vi "Launch Event Reporter.vi"(8 "error in (no error)":errorcluster, 11 "Volatus Core in":refnum<class "Volatus Core.lvclass">) -> (0 "error out":errorcluster, 3 "Volatus Core out":refnum<class "Volatus Core.lvclass">)   [LabVIEW 2020, in "Volatus.lvlib" / "Volatus Core.lvclass"]
uses:
  Volatus Core.lvclass
  C:/dev/lv20CE/relink/lv-volatus/Volatus/Module/Module.lvclass
  VolatusConfig/VolatusConfigElement/VolatusConfigElement.lvclass
  Module/Module.lvclass/Module.ctl
  VolatusConfig/VolatusConfigElement/VolatusConfigElement.lvclass/VolatusConfigElement.ctl
  VolatusAPI/VolatusAPI.lvclass/VolatusAPI.ctl
  Volatus Core.lvclass/Volatus Core.ctl
  VolatusConfig/VolatusConfigElement/Element.vi
  MessageQ/MessageQ.lvclass
  Module/Module.lvclass
  VolatusAPI/VolatusAPI.lvclass
  VectoEventBridge/VectoEventBridge.lvclass
  Event Reporter Module/Event Reporter Module.lvclass
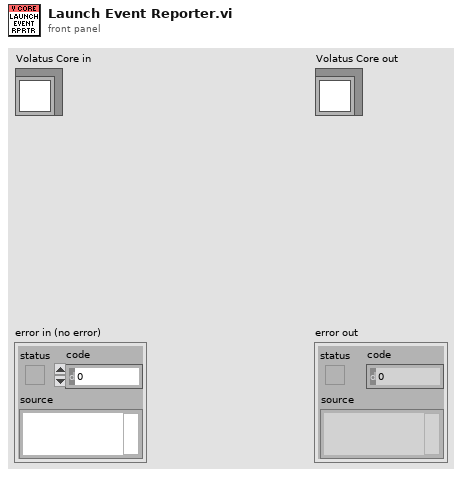
[diagram p1: front panel]
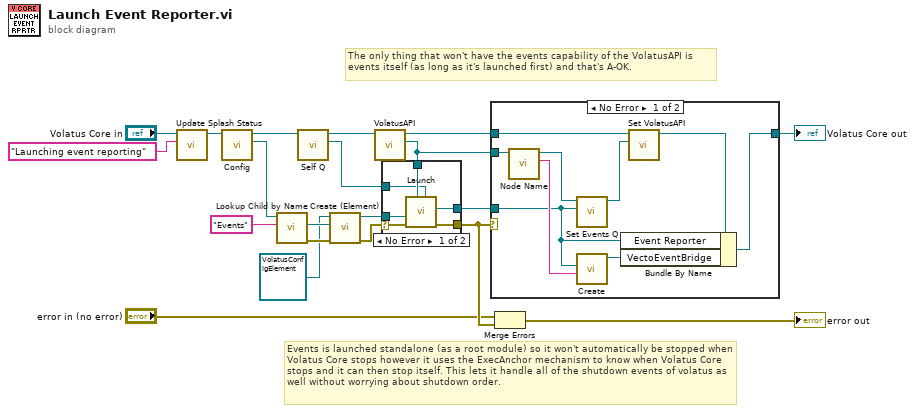
[diagram p0: block diagram]
diagram:
  # "Events is launched standalone (as a root module) so it won't automatically be stopped when Volatus Core stops however it uses the ExecAnchor mechanism to know when Volatus Core stops and it can then stop itself. This lets it handle all of the shutdown events of volatus as well without worrying about shutdown order."
  # "The only thing that won't have the events capability of the VolatusAPI is events itself (as long as it's launched first) and that's A-OK."
  n1 = call "Update Splash Status.vi"("Status"="Launching event reporting", "Volatus Core in"="Volatus Core in") -> ("Volatus Core out"=w2:refnum<class "Volatus Core.lvclass">)  [unwired: 8 in, 1 out]
  n2 = call "Config.vi"("Module in"=w2) -> ("Config"=w19:refnum<class "VolatusConfigElement.lvclass">, "Module out"=w7:refnum<class "Volatus Core.lvclass">)  [unwired: 9 in]
  n3 = call "Lookup Child by Name.vi"("Child Name"="Events" ("Name"), "VolatusConfigElement in"=w19) -> ("error out"=w12:errorcluster, "Child"=w11:refnum<class "Config Element.lvclass">)  [unwired: 6 in, 2 out]
  n4 = call "Self Q.vi"("Module in"=w7) -> ("Self Q"=w3:refnum<class "MessageQ.lvclass">, "Module out"=w4:refnum<class "Volatus Core.lvclass">)  [unwired: 9 in]
  n5 = call "Create (Element).vi"("error in (no error)"=w12, "Element"=w11, "VolatusConfigElement in"=refnum<class "VolatusConfigElement.lvclass"> refnum) -> ("error out"=w10:errorcluster, "VolatusConfigElement out"=w9:refnum<class "VolatusConfigElement.lvclass">)  [unwired: 7 in]
  n6 = call "VolatusAPI.vi"("Module in"=w4) -> ("VolatusAPI"=w5:refnum<class "VolatusAPI.lvclass">, "Module out"=w6:refnum<class "Volatus Core.lvclass">)  [unwired: 9 in]
  n7 = case shown="No Error" w10 {
    selector: w10 -> [w24 w27]
    tunnel: w9 -> [w23 _]
    tunnel: [w25 _] -> w17
    tunnel: [w26 w27] -> w15
    tunnel: w5 -> [w22 _]
    tunnel: w3 -> [w21 _]
    frame No Error {
      n8 = call "Launch.vi"("Status Q"=w21, "VolatusAPI"=w22, "error in (no error)"=w24, "Config"=w23) -> ("error out"=w26:errorcluster, "MessageQ"=w25:refnum<class "MessageQ.lvclass">)  [unwired: 6 in]
    }
    frame Error {
    }
  }
  n9 = case shown="No Error" w15 {
    tunnel: w17 -> [w28 _]
    tunnel: w6 -> [w36 w37]
    tunnel: [w33 w37] -> w16
    tunnel: w5 -> [w29 _]
    frame No Error {
      n10 = call "Node Name.vi"("VolatusAPI in"=w29) -> ("Node Name"=w30:string, "VolatusAPI out"=w31:refnum<class "VolatusAPI.lvclass">)  [unwired: 8 in, 1 out]
      n11 = call "Set Events Q.vi"("Events Q"=w28, "VolatusAPI in"=w31) -> ("VolatusAPI out"=w35:refnum<class "VolatusAPI.lvclass">)  [unwired: 9 in]
      n12 = call "Create.vi"("Node"=w30, "MsgQ"=w28) -> ("VectoEventBridge out"=w32:refnum<class "VectoEventBridge.lvclass">)  [unwired: 8 in, 1 out]
      n13 = call "Set VolatusAPI.vi"("VolatusAPI"=w35, "Module in"=w36) -> ("Module out"=w34:refnum<class "Volatus Core.lvclass">)  [unwired: 9 in]
      n14 = Bundle By Name(cluster=w34, "Event Reporter"=w28, "VectoEventBridge"=w32) -> (w33:refnum<class "Volatus Core.lvclass">)
    }
    frame Error {
    }
  }
  "Volatus Core out" <- w16
  n15 = Merge Errors("error in (no error)", w15) -> (→"error out":errorcluster)
